vi "Project List.vi"(7 "Project Store in":refnum<class "Project Store.lvclass">, 8 "error in":errorcluster) -> (0 "error out":errorcluster, 2 "Project IDs":string[](array[string]), 3 "Project Names":string[](array[string]), 5 "Project Store out":refnum<class "Project Store.lvclass">)   [LabVIEW 2026]
doc: "Returns the active projects of the Project Store in Sort Order, as the parallel arrays a ring or listbox needs: Project Names for display and Project IDs to look up the selection. Inactive projects are left out.\n\nInputs: Project Store in (Project Store or a child such as Project Store-INI, already read from its data source); error in.\nOutputs: Project Names; Project IDs (same order as Project Names); Project Store out; error out.\n\nGenerated by: Claude"
uses:
  Storage/Project Store/Project Store.lvclass
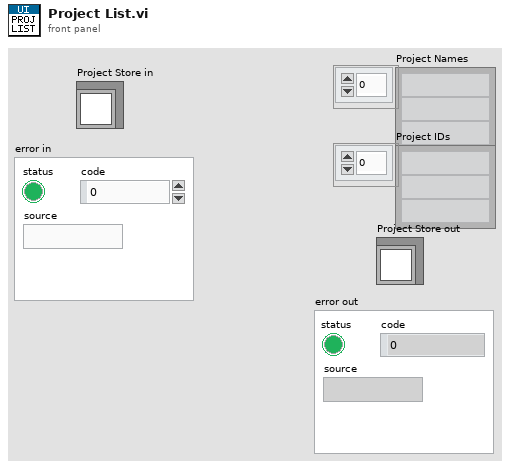
[diagram p1: front panel]
types:
  T1 = typedef "Project List.ctl" = T2[]
  T2 = typedef "Project.ctl" = cluster{"ID":string, "Name":string, "Active":bool, "Sort Order":i32}
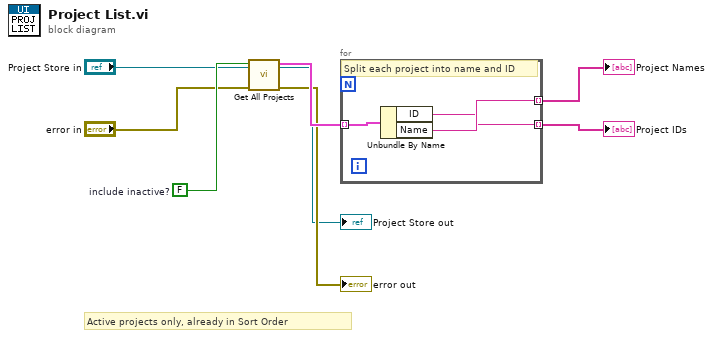
[diagram p0: block diagram]
diagram:
  w7 = FALSE  # include inactive?
  # "Active projects only, already in Sort Order"
  n1 = call-dynamic "Get All Projects.vi"("Project Store in"="Project Store in", "error in (no error)"="error in", "include inactive?"=w7) -> ("error out"=→"error out":errorcluster, "Projects"=w8:T1, "Project Store out"=→"Project Store out":refnum<class "Project Store.lvclass">)  [unwired: 6 in]
  n2 = for {
    tunnel: w8 -> [w9] mode=indexing
    tunnel: [w11] -> w3 mode=indexing
    tunnel: [w10] -> w4 mode=indexing
    # "Split each project into name and ID"
    n3 = Unbundle By Name(w9) -> ("ID"=w10:string, "Name"=w11:string)
  }
  "Project Names" <- w3
  "Project IDs" <- w4
